vi "Create Host Key Database Refnum.vi"(8 "error in (no error)":errorcluster, 11 "LIBSSH2_KNOWNHOSTS*":u64 format="%.0x") -> (0 "error out":errorcluster, 3 "host key database":T1)   [LabVIEW 2017, in "libssh2.lvlib"]
uses:
  libssh2.lvlib
  Host Key Database Refnum.ctl
  Host Key Database Refnum Data.ctl
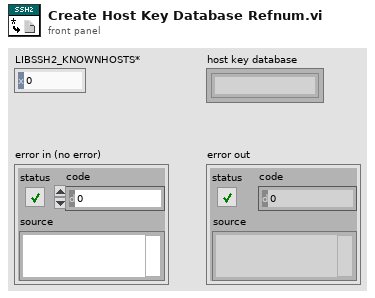
[diagram p1: front panel]
types:
  T1 = typedef "libssh2.lvlib/Host Key Database Refnum.ctl" = refnum<k1>
  T2 = typedef "libssh2.lvlib/Host Key Database Refnum Data.ctl" = cluster{"LIBSSH2_KNOWNHOSTS*":u64, "semaphore":T3}
  T3 = typedef "Semaphore RefNum" = refnum<k1>
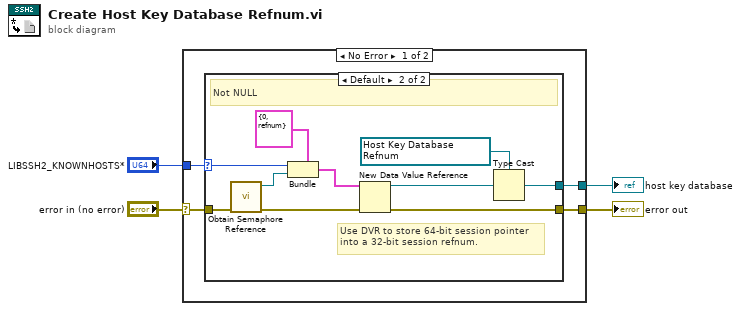
[diagram p0: block diagram]
diagram:
  n1 = case shown="No Error" "error in (no error)" {
    selector: "error in (no error)" -> [w6 w20]
    tunnel: [w8 _] -> w4
    tunnel: [w7 w20] -> w3
    tunnel: "LIBSSH2_KNOWNHOSTS*" -> [w5 _]
    frame No Error {
      n2 = case shown="Default" w5 {
        selector: w5 -> [_ w17]
        tunnel: [_ w18] -> w8
        tunnel: [w9 w15] -> w7
        tunnel: w6 -> [w9 w12]
        frame 0 {
          # "NULL"
        }
        frame Default {
          w19 = T1 refnum items=["host key database"] ("known hosts collection")
          # "Use DVR to store 64-bit session pointer\ninto a 32-bit session refnum."
          # "Not NULL"
          n3 = call <vilib>:"Obtain Semaphore Reference.vi"("error in (no error)"=w12) -> ("error out"=w11:errorcluster, "semaphore"=w10:T3)  [unwired: 4 in, 1 out]
          n4 = Bundle(cluster=T2 {"LIBSSH2_KNOWNHOSTS*"=0, "semaphore"=refnum} ("host key database data"), "LIBSSH2_KNOWNHOSTS*"=w17, "semaphore"=w10) -> (w14:T2)
          n5 = New Data Value Reference(data value=w14, error in=w11) -> (data value reference=w16:refnum<data-value>, error out=w15:errorcluster)
          n6 = Type Cast(type=w19, x=w16) -> (*(type *) &x=w18:T1)
        }
      }
    }
    frame Error {
    }
  }
  "host key database" <- w4
  "error out" <- w3
